vi "from_item.vi"(8 "error in (no error)":errorcluster, 10 "item_ref":u64) -> (0 "error out":errorcluster, 3 "Table out":refnum<class "Table.lvclass">)   [LabVIEW 2020, in "toml_edit.lvlib" / "Table.lvclass"]
uses:
  Table.lvclass
  Table.lvclass/Table.ctl
  Item/Item.lvclass
  dragon_toml_64.dll
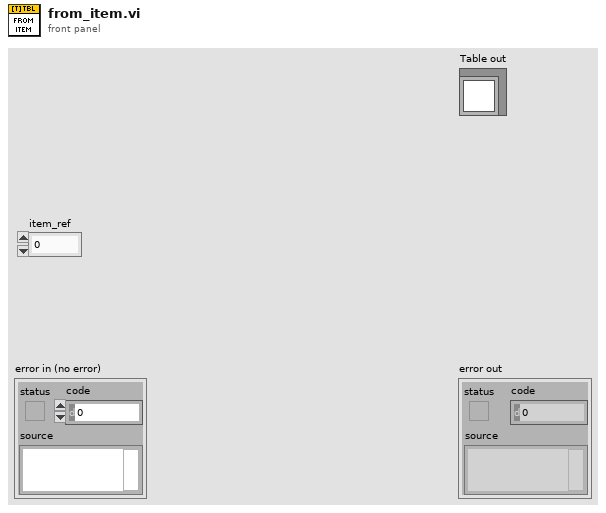
[diagram p1: front panel]
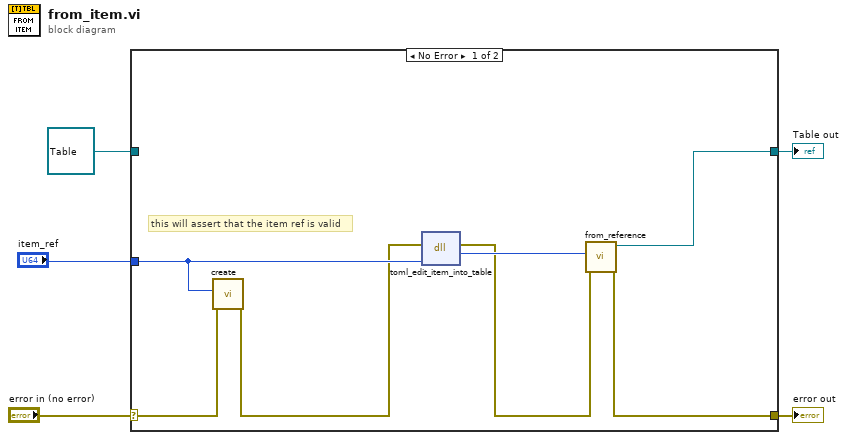
[diagram p0: block diagram]
diagram:
  n1 = case shown="No Error" "error in (no error)" {
    selector: "error in (no error)" -> [w11 w14]
    tunnel: [w6 w14] -> w4
    tunnel: [w8 w13] -> w2
    tunnel: refnum<class "Table.lvclass"> refnum ("Table in") -> [_ w13]
    tunnel: "item_ref" -> [w12 _]
    frame No Error {
      # "this will assert that the item ref is valid"
      n2 = call "create.vi"("error in (no error)"=w11, "ref"=w12) -> ("error out"=w10:errorcluster)  [unwired: 7 in, 2 out]
      n3 = dll-call lib="C:/projects/dragon-desktop/source/submodules/toml-edit-labview/lv_src/dragon_toml_*.*" fn="toml_edit_item_into_table"(error in=w10, "item_ref"=w12) -> (error out=w7:errorcluster, "table_ref"=w9:u64)  [unwired: 3 in, 1 out]
      n4 = call "from_reference.vi"("error in (no error)"=w7, "ref"=w9) -> ("error out"=w6:errorcluster, "Table out"=w8:refnum<class "Table.lvclass">)  [unwired: 8 in]
    }
    frame Error {
    }
  }
  "error out" <- w4
  "Table out" <- w2
